vi "ParseResponseStatus.vi"(8 "error in (no error)":errorcluster, 10 "Headers":string) -> (0 "error out":errorcluster, 1 "StatusText":string, 2 "StatusCode":i32)   [LabVIEW 2017]
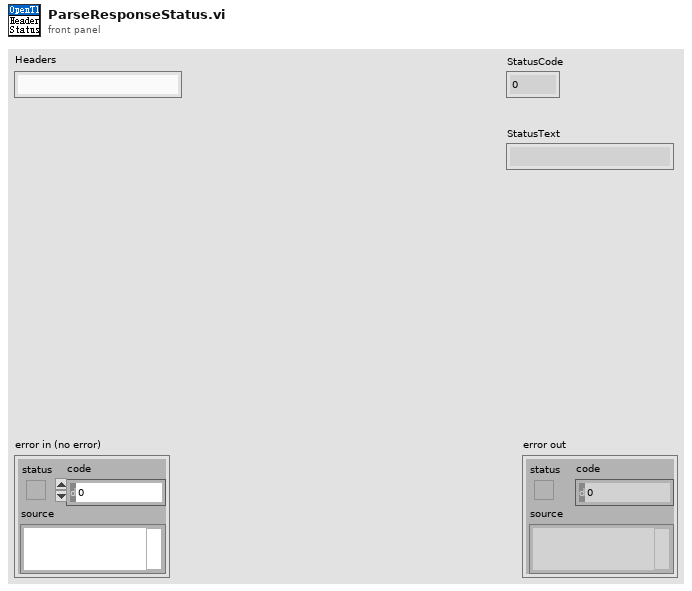
[diagram p1: front panel]
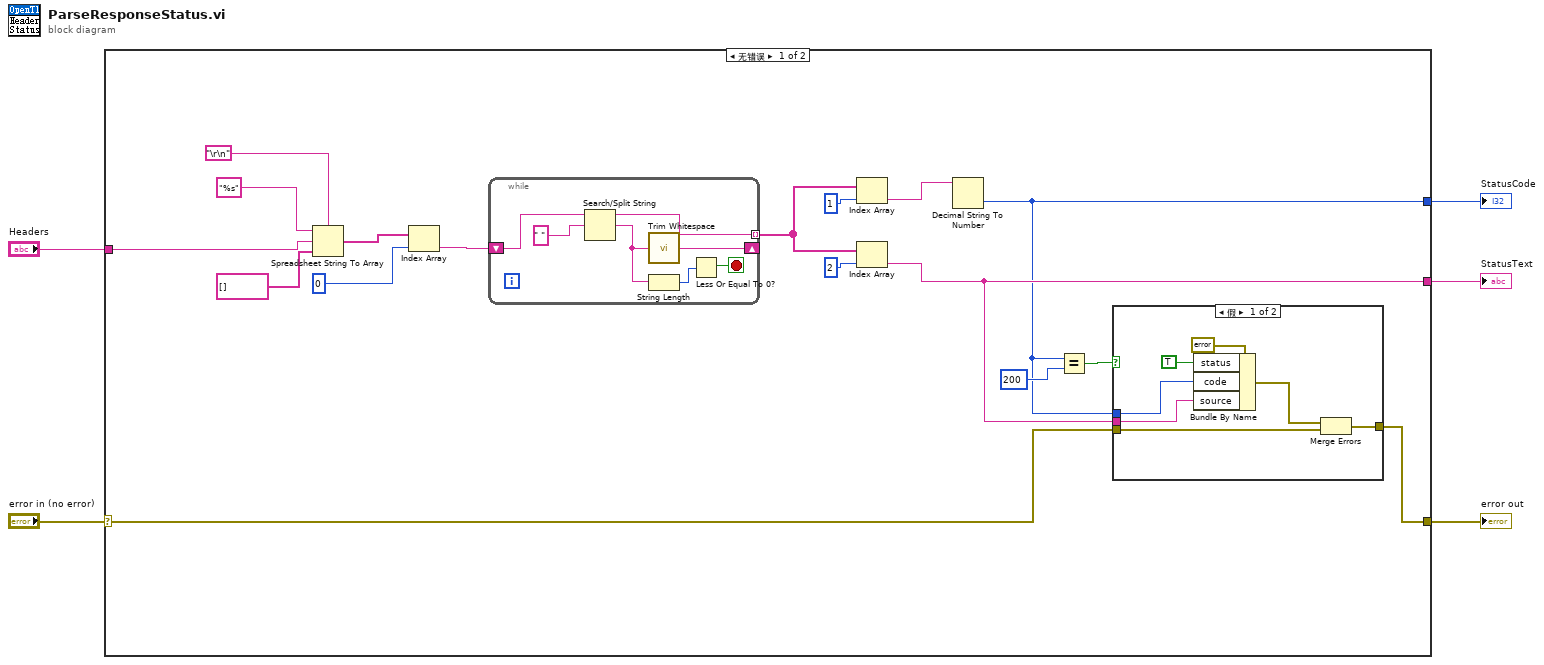
[diagram p0: block diagram]
diagram:
  n1 = case shown="无错误" "error in (no error)" {
    selector: "error in (no error)" -> [w8 w38]
    tunnel: [w6 w38] -> w4
    tunnel: "Headers" -> [w12 _]
    tunnel: [w9 _] -> w2
    tunnel: [w7 _] -> w1
    frame No Error {
      n2 = Spreadsheet String To Array(delimiter (Tab)="\r\n", format string="%s", spreadsheet string=w12, array type (2D Dbl)=string[] []) -> (array=w18:string[])
      n3 = Index Array(array=w18, index=0 ("索引")) -> (element=w17:string)
      n4 = while {
        shift-right: [w34] -> _
        shift-left: w17 -> [w37]
        tunnel: [w35] -> w14 mode=indexing
        stop <- w31 stop-if-true
        n5 = Search/Split String(string=w37, search string/char (-)=" " ("搜索字符串/字符(-)")) -> (substring before match=w35:string, match + rest of string=w32:string)  [unwired: 1 in, 1 out]
        n6 = call <vilib>:"Trim Whitespace.vi"("string"=w32) -> ("trimmed string"=w34:string)  [unwired: 1 in]
        n7 = String Length(string=w32) -> (length=w33:i32)
        n8 = Less Or Equal To 0?(x=w33) -> (x <= 0?=w31:bool)
      }
      n9 = Index Array(array=w14, index=1 ("索引")) -> (element=w13:string)
      n10 = Index Array(array=w14, index=2 ("索引")) -> (element=w9:string)
      n11 = Decimal String To Number(string=w13) -> (number=w7:i32)  [unwired: 2 in, 1 out]
      n12 = Equal?(x=w7, y=200) -> (x = y?=w10:bool)
      n13 = case shown="假" w10 {
        tunnel: [w26 w30] -> w6
        tunnel: w8 -> [w24 w30]
        tunnel: w9 -> [w27 _]
        tunnel: w7 -> [w28 _]
        frame False {
          n14 = Bundle By Name(cluster=errorcluster {"status"=FALSE, "code"=0, "source"=""} ("error in (no error)"), "status"=TRUE, "code"=w28, "source"=w27) -> (w25:errorcluster)
          n15 = Merge Errors(w25, w24) -> (w26:errorcluster)
        }
        frame True {
        }
      }
    }
    frame Error {
    }
  }
  "error out" <- w4
  "StatusText" <- w2
  "StatusCode" <- w1
